vi "VHistory - History Controller.vi"(4 "value condition":T2 {"Range_Max" format="%.2f"; "Range_Min" format="%.2f"; "Delta" format="%.2f"}, 6 "time conditions":cluster{"Step, ms":u32, "Gate, ms":u32}, 7 "VC Handle":T4=-1, 8 "error in":errorcluster, 9 "cmd (nop:default)":T3(ring), 10 "history length":i32, 11 "name_spec":string) -> (0 "error out":errorcluster, 1 "more data":cluster{"store Writer IDs":bool}, 2 "history info":T1 {"oldest timestamp" format="%<%H:%M:%S%2u\n%d/%m/%Y>T"; "NewVals mode"."last read time" format="%<%H:%M:%S%2u\n%d/%m/%Y>T"; "newest timestamp" format="%<%H:%M:%S%2u\n%d/%m/%Y>T"}, 3 "dup name_spec":string)   [LabVIEW 2021]
doc: "This VI controls and monitors the status of variable histories. Refer to the VI help for more details.\n\n<b>VC Handle</b> specifies the handle of the variable context. To operate on a global variable, pass -1 to this input. This input is ignored if the <b>name_spec</b> control refers to a variable by an alias.\n\n<b>name_spec</b> is the name specifier of the desired variable. Usually, it is merely a variable name; however, its generic format is '[name][=alias]', where either 'name' or '=alias' can be omitted but not both.\n\n<b>history length</b> control specifies the maximum number of values that a history can store. A history is arranged as a circular buffer and can contain as many recent values as specified during its creation. This control is only used when the VI creates a variable history.\n\n<b>cmd</b> control specifies the action to be performed. Possible actions are:\n 'create' : creates a history and attaches it to the given variable (without storing writer ID for values).\n 'destroy' : destroys the history.\n 'reset' : removes all values from the history.\n 'get info' : returns the history parameters in the <b>history info</b> indicator.\n 'config' : sets new time conditions and value conditions for the history.\n 'create_wrid' : identical to the 'create' action, but it also causes the history to store <b>writer ID</b> for each stored value.\n\n<b>time conditions</b> cluster is an optional control to specify the time conditions used to maintain the variable history.\n\n<b>value condition</b> cluster is an optional control to specify the value condition used to maintain the variable history.\n\n<b>history info</b> indicator returns information about both the configuration and state of the history.\n\n<b>more data</b> indicator is a cluster containing only the <b>store Writer IDs</b> member, which indicates whether the history stores writer IDs.\n\n::: CalcExpress Toolkit :::\nCopyright (c) 2000-2026 Konstantin Shifershteyn. All rights reserved."
uses:
  cetypes.llb/VarMan Variable Context Handle.ctl
  cetypes.llb/VarMan History Info.ctl
  cetypes.llb/VarMan Error Code.ctl
  cersrc/celveng32.dll
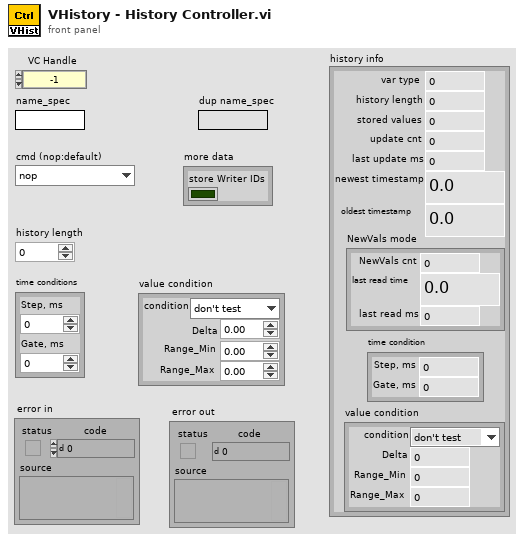
[diagram p1: front panel]
types:
  T1 = typedef "VarMan History Info.ctl" = cluster{"var type":u32, "history length":u32, "stored values":u32, "update cnt":u32, "last update ms":u32, "newest timestamp":dbl, "oldest timestamp":dbl, "NewVals mode":cluster{"NewVals cnt":u32, "last read time":dbl, "last read ms":u32}, "time condition":cluster{"Step, ms":u32, "Gate, ms":u32}, "value condition":cluster{"condition":enum32{"don't test", "changed", "abs deviation", "rel deviation", "out of range", "within range"}, "Delta":dbl, "Range_Min":dbl, "Range_Max":dbl}}
  T2 = cluster{"condition":enum32{"don't test", "changed", "abs deviation", "rel deviation", "out of range", "within range"}, "Delta":dbl, "Range_Min":dbl, "Range_Max":dbl}
  T3 = enum32{"nop", "create", "destroy", "reset", "get info", "config", "create_wrid"}
  T4 = typedef "VarMan Variable Context Handle.ctl" = i32
  T5 = typedef "VarMan Error Code.ctl" = u16
  T6 = enum32{"don't test", "changed", "abs deviation", "rel deviation", "out of range", "within range"}
  T7 = cluster{"history length":i32, "Step, ms":u32, "Gate, ms":u32, "condition":enum32{"don't test", "changed", "abs deviation", "rel deviation", "out of range", "within range"}, "Delta":dbl, "Range_Min":dbl, "Range_Max":dbl}
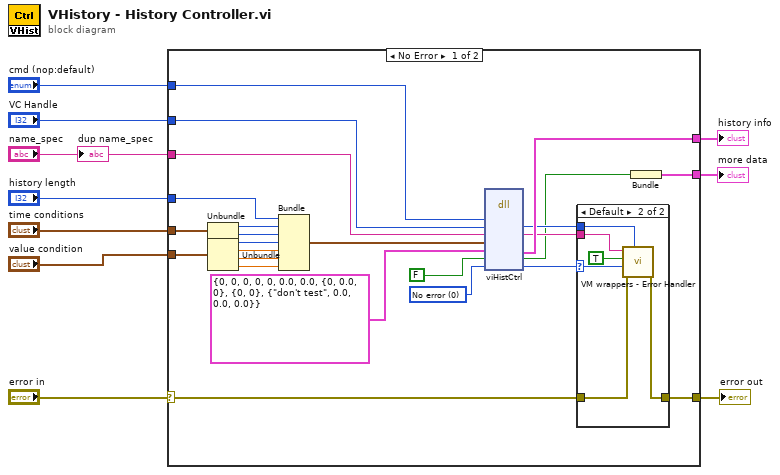
[diagram p0: block diagram]
diagram:
  n1 = case shown="No Error" "error in" {
    selector: "error in" -> [w13 w42]
    tunnel: [w34 w42] -> w10
    tunnel: "VC Handle" -> [w33 _]
    tunnel: "name_spec" -> [w32 _]
    tunnel: [w31 _] -> w7
    tunnel: "cmd (nop:default)" -> [w28 _]
    tunnel: "time conditions" -> [w27 _]
    tunnel: "value condition" -> [w26 _]
    tunnel: "history length" -> [w19 _]
    tunnel: [w11 _] -> w1
    frame No Error {
      w29 = T5 0 items=["No error", "Invalid variable type", "Variable not found", "Variable already exists", "Invalid context handle", "Input error", "Invalid data format", "No history attached", "History already attached", "Invalid history parameters", "Wrong variable name", "Wrong alias name", "Non-unique alias", "Alias not found", "No alias associated", "Alias already associated", "Wrong context name", "Non-unique context name", "Context name not found", "Invalid parameter", "Generic error", "Memory Full", "Unrecognized LV error", "Unknown error code"] ("VarMan error")
      n2 = Unbundle(w27) -> ("Step, ms"=w20:u32, "Gate, ms"=w21:u32)
      n3 = Unbundle(w26) -> ("condition"=w22:T6, "Delta"=w23:dbl, "Range_Min"=w24:dbl, "Range_Max"=w25:dbl)
      n4 = Bundle("history length"=w19, "Step, ms"=w20, "Gate, ms"=w21, "condition"=w22, "Delta"=w23, "Range_Min"=w24, "Range_Max"=w25) -> (w18:T7)  [unwired: 1 in]
      n5 = dll-call lib="C:/LV Projects/CalcExpress 40 LV2021/vi.lib/addons/CalcExpress/cersrc/celveng*.dll" fn="viHistCtrl"("cmd"=w28, "vch"=w33, "name"=w32, "histPars"=w18, "histInfo"=T1 {"var type"=0, "history length"=0, "stored values"=0, "update cnt"=0, "last update ms"=0, "newest timestamp"=0.0, "oldest timestamp"=0.0, "NewVals mode"={"NewVals cnt"=0, "last read time"=0.0, "last read ms"=0}, "time condition"={"Step, ms"=0, "Gate, ms"=0}, "value condition"={"condition"=enum."don't test", "Delta"=0.0, "Range_Min"=0.0, "Range_Max"=0.0}} ("history info"), "hasWrID"=FALSE, "errc"=w29) -> ("vch"=w14:i32, "name"=w15:string, "histInfo"=w31:T1, "hasWrID"=w12:bool, "errc"=w17:T5)  [unwired: 6 in, 2 out]
      n6 = case shown="Default" w17 {
        selector: w17 -> [_ w38]
        tunnel: w13 -> [w35 w41]
        tunnel: [w35 w40] -> w34
        tunnel: w15 -> [_ w37]
        tunnel: w14 -> [_ w36]
        frame 0 {
        }
        frame Default {
          n7 = call "VM wrappers - Error Handler.vi"("VC Handle"=w36, "error before"=w41, "VarMan error"=w38, "show name spec (F)"=TRUE, "name spec"=w37) -> ("error out"=w40:errorcluster)  [unwired: 5 in, 1 out]
        }
      }
      n8 = Bundle("hasWrID"=w12) -> (w11:cluster{"hasWrID":bool})  [unwired: 1 in]
    }
    frame Error {
    }
  }
  "error out" <- w10
  "history info" <- w7
  "more data" <- w1
  "dup name_spec" <- "name_spec"
